vi "Dernier_element_2D.vi"(0 "Programme":cluster{"chaîne":string, "Valeur":dbl}[][](array[cluster]) {"Valeur" format="%#.1f"}) -> (1 "Dernier segment":cluster{"chaîne":string, "Valeur":dbl}[](array[cluster]) {"Valeur" format="%#.1f"}, 2 "Indice N":i32, 3 "Taille/Indice N+1":i32)   [LabVIEW 2022 SP3]
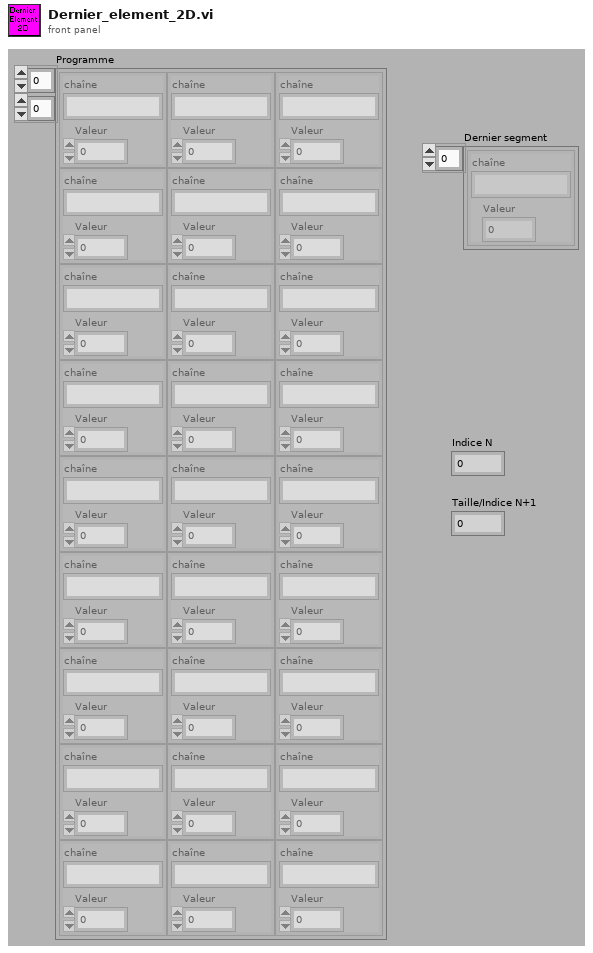
[diagram p1: front panel]
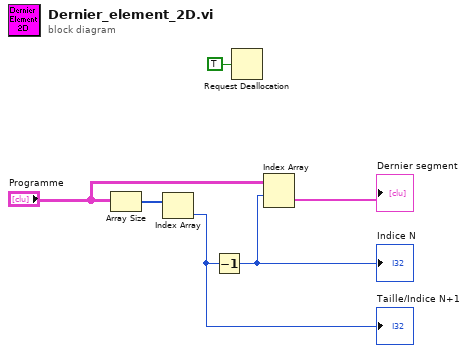
[diagram p0: block diagram]
diagram:
  n1 = Array Size(array="Programme") -> (size(s)=w5:i32[])
  n2 = Index Array(array=w5) -> (element=w4:i32)  [unwired: 1 in]
  "Taille/Indice N+1" <- w4
  n3 = Decrement(x=w4) -> (x-1=w6:i32)
  "Indice N" <- w6
  n4 = Request Deallocation(TRUE ("flag")) -> ()
  n5 = Index Array(array="Programme", index (row)=w6) -> (element=→"Dernier segment":cluster{"chaîne":string, "Valeur":dbl}[])  [unwired: 1 in]
